vi "RPC Method ThermalChamberController SubscribeChamberStatusUpdated.vi"(8 "error in (no error)":errorcluster, 11 "gRPC service in":refnum<class "ThermalChamberController.lvclass">) -> (0 "error out":errorcluster, 3 "gRPC service out":refnum<class "ThermalChamberController.lvclass">)   [LabVIEW 2020, in "thermal-chamber-controller_server.lvlib" / "ThermalChamberController.lvclass"]
uses:
  ThermalChamberController.lvclass
  support/Stream Data--cluster.ctl
  <vilib>/gRPC/LabVIEW gRPC Library/Shared/grpcId.ctl
  ThermalChamberController.lvclass/ThermalChamberController.ctl
  <vilib>/gRPC/LabVIEW gRPC Library/grpc-lvsupport-release.lvlib
  Program Files (x86)/National Instruments/LabVIEW 2020/examples/DQMH Consortium/DQMH Fundamentals - Thermal Chamber/Libraries/Thermal Chamber Controller_DQMH/Thermal Chamber Controller_DQMH.lvlib
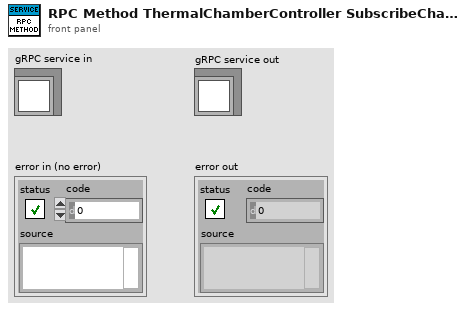
[diagram p1: front panel]
types:
  T1 = typedef "Stream Data--cluster.ctl" = cluster{"gRPCid":T2, "Active":bool, "timeout":i32}
  T2 = typedef "grpc-lvsupport-release.lvlib/grpcId.ctl" = u64
  T3 = typedef "thermal-chamber-controller_server.lvlib/ThermalChamberController.lvclass/Server Internal UEs.ctl" = cluster{"ThermalChamberController StartModule Internal UE":refnum<user-event>, "ThermalChamberController ShowModulePanel Internal UE":refnum<user-event>, "ThermalChamberController HideModulePanel Internal UE":refnum<user-event>, "ThermalChamberController StopModule Internal UE":refnum<user-event>, "ThermalChamberController UpdateSetPoint Internal UE":refnum<user-event>, "ThermalChamberController UpdateRampRate Internal UE":refnum<user-event>, "ThermalChamberController UpdateHeaterState Internal UE":refnum<user-event>, "ThermalChamberController SubscribeChamberStatusUpdated Internal UE":refnum<user-event>, "ThermalChamberController SubscribeSetPointUpdated Internal UE":refnum<user-event>, "ThermalChamberController SubscribeRampRateUpdated Internal UE":refnum<user-event>, "ThermalChamberController SubscribeHeaterStateUpdated Internal UE":refnum<user-event>}
  T4 = typedef "thermal-chamber-controller_server.lvlib/ThermalChamberController.lvclass/Server gRPC UEs.ctl" = cluster{"ThermalChamberController StartModule gRPC UE":refnum<user-event>, "ThermalChamberController ShowModulePanel gRPC UE":refnum<user-event>, "ThermalChamberController HideModulePanel gRPC UE":refnum<user-event>, "ThermalChamberController StopModule gRPC UE":refnum<user-event>, "ThermalChamberController UpdateSetPoint gRPC UE":refnum<user-event>, "ThermalChamberController UpdateRampRate gRPC UE":refnum<user-event>, "ThermalChamberController UpdateHeaterState gRPC UE":refnum<user-event>, "ThermalChamberController SubscribeChamberStatusUpdated gRPC UE":refnum<user-event>, "ThermalChamberController SubscribeSetPointUpdated gRPC UE":refnum<user-event>, "ThermalChamberController SubscribeRampRateUpdated gRPC UE":refnum<user-event>, "ThermalChamberController SubscribeHeaterStateUpdated gRPC UE":refnum<user-event>}
  T5 = typedef "Thermal Chamber Controller_DQMH.lvlib/Broadcast Events--cluster.ctl" = cluster{"Module Did Init":refnum<user-event>, "Status Updated":refnum<user-event>, "Error Reported":refnum<user-event>, "Module Did Stop":refnum<user-event>, "Update Module Execution Status":refnum<user-event>, "Chamber Status Updated":refnum<user-event>, "Set Point Updated":refnum<user-event>, "Ramp Rate Updated":refnum<user-event>, "Heater State Updated":refnum<user-event>}
  T6 = typedef "Thermal Chamber Controller_DQMH.lvlib/Heater State--enum.ctl" = enum16{"Heater Enabled", "Heater Disabled"}
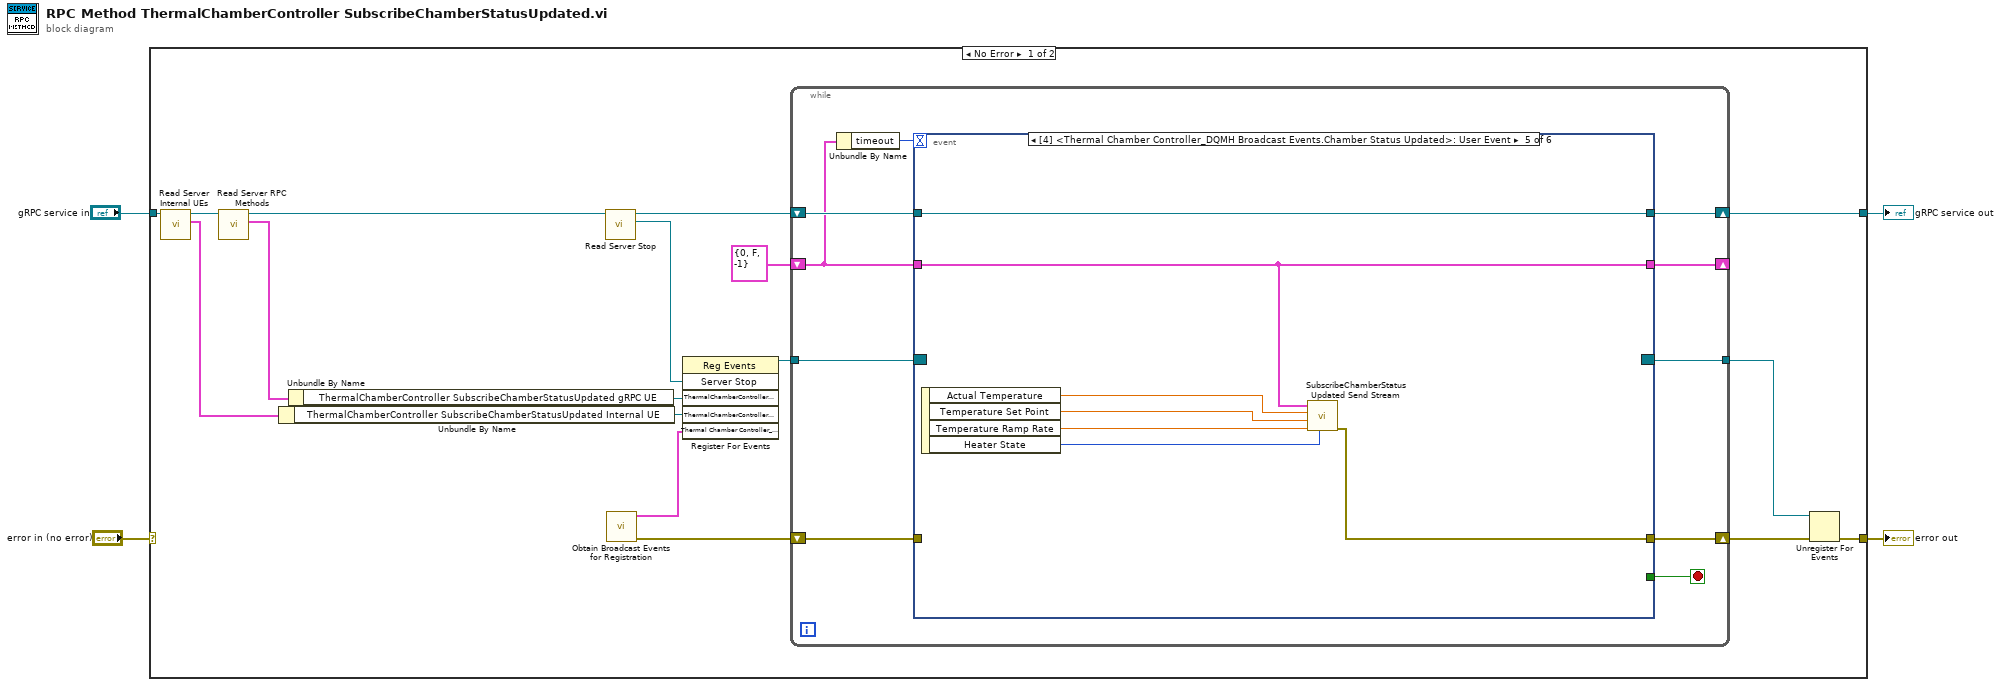
[diagram p0: block diagram]
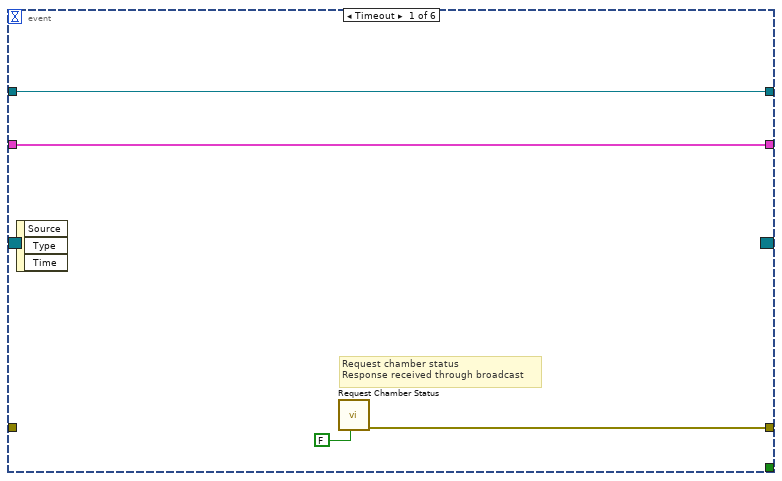
[diagram p2: hidden frame]
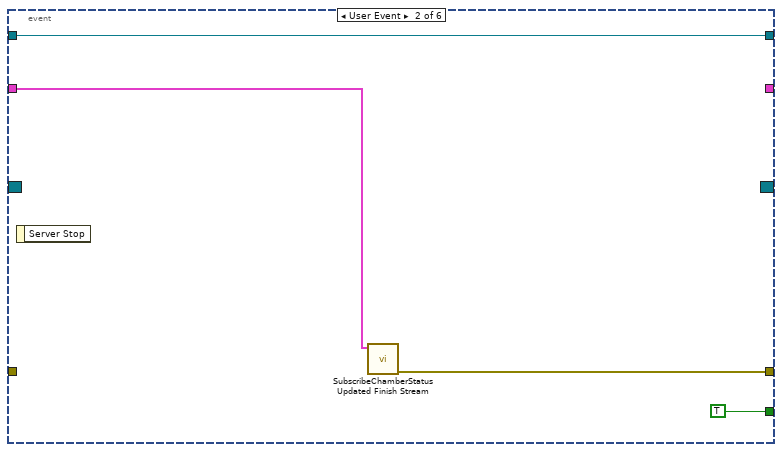
[diagram p3: hidden frame]
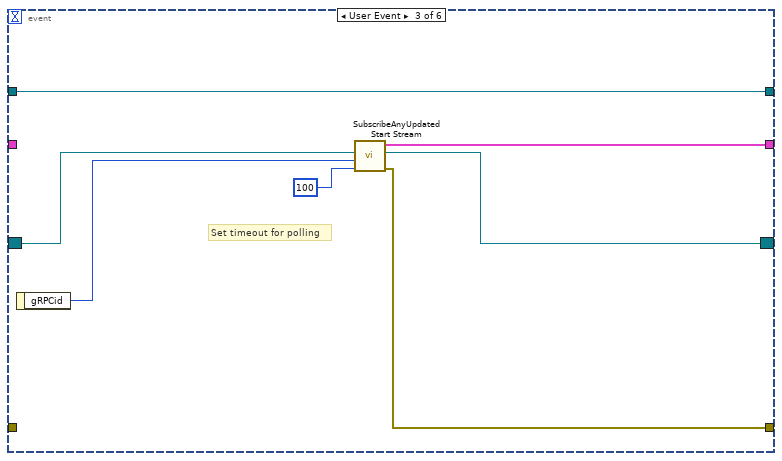
[diagram p4: hidden frame]
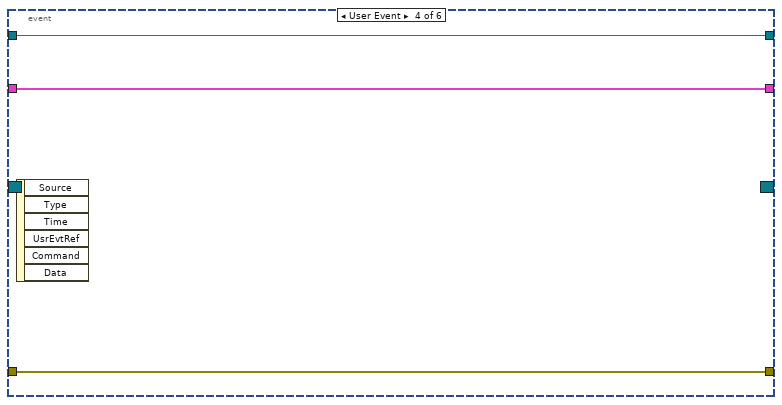
[diagram p5: hidden frame]
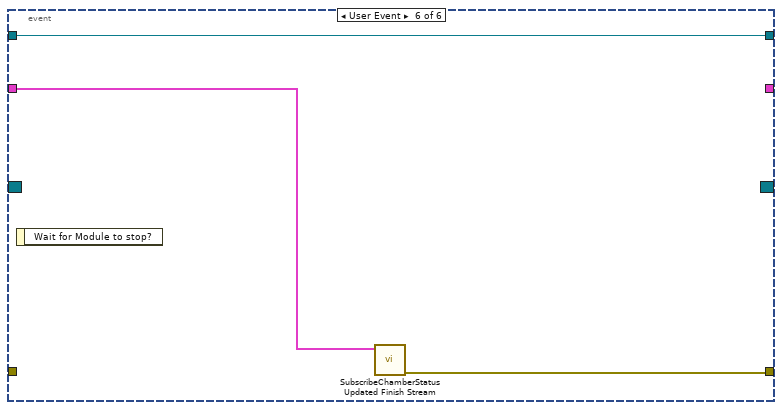
[diagram p6: hidden frame]
diagram:
  n1 = case shown="No Error" "error in (no error)" {
    selector: "error in (no error)" -> [_ w61]
    tunnel: [w16 w61] -> w3
    tunnel: "gRPC service in" -> [w19 w60]
    tunnel: [w8 w60] -> w1
    frame No Error {
      n2 = call "Read Server Internal UEs.vi"("gRPC service in"=w19) -> ("Server Internal UEs"=w12:T3, "gRPC service out"=w18:refnum<class "ThermalChamberController.lvclass">)  [unwired: 8 in, 1 out]
      n3 = call "Read Server RPC Methods.vi"("gRPC service in"=w18) -> ("Server RPC Methods"=w14:T4, "gRPC service out"=w9:refnum<class "ThermalChamberController.lvclass">)  [unwired: 8 in, 1 out]
      n4 = Unbundle By Name ("Unbundle Internal UE")(w12) -> ("ThermalChamberController SubscribeChamberStatusUpdated Internal UE"=w11:refnum<user-event>)
      n5 = Unbundle By Name ("Unbundle gRPC UE")(w14) -> ("ThermalChamberController SubscribeChamberStatusUpdated gRPC UE"=w13:refnum<user-event>)
      n6 = call-dynamic "Read Server Stop.vi"("gRPC service in"=w9) -> ("Server Stop"=w21:refnum<user-event>, "gRPC service out"=w10:refnum<class "ThermalChamberController.lvclass">)  [unwired: 8 in, 1 out]
      n7 = call "Obtain Broadcast Events for Registration.vi"() -> ("error out"=w6:errorcluster, "Thermal Chamber Controller_DQMH Broadcast Events"=w5:T5)  [unwired: 9 in, 1 out]
      n8 = register-events(w21, w13, w11, w5) -> (reference out=w20:refnum<event-registration>)  [unwired: 2 in, 1 out]
      n9 = while {
        tunnel: w20 -> [w31]
        tunnel: [w27] -> w15
        shift-right: [w28] -> w17
        shift-left: w6 -> [w29]
        shift-right: [w25] -> w8
        shift-left: w10 -> [w26]
        shift-right: [w24] -> _
        shift-left: T1 {"gRPCid"=0, "Active"=FALSE, "timeout"=-1} ("Stream Data") -> [w23]
        stop <- w30 stop-if-true
        n10 = Unbundle By Name(w23) -> ("timeout"=w22:i32)
        n11 = event "RPC Method Event Structure" shown="[4] <Thermal Chamber Controller_DQMH Broadcast Events.Chamber Status Updated>: User Event" {
          selector: w31 -> [_ _ w44 _ _ _]
          dyn-events: [_ _ w42 _ _ _] -> w27
          timeout: w22 -> [_ _ _ _ _ _]
          tunnel: [_ TRUE _ _ _ _] -> w30
          tunnel: w29 -> [_ _ _ w49 _ _]
          tunnel: [w32 w37 w41 w49 w50 w57] -> w28
          tunnel: w26 -> [w35 w38 w46 w48 w56 w59]
          tunnel: [w35 w38 w46 w48 w56 w59] -> w25
          tunnel: w23 -> [w34 w36 _ w47 w55 w58]
          tunnel: [w34 _ w45 w47 w55 _] -> w24
          event Timeout {
            # "Request chamber status\nResponse received through broadcast"
            n12 = event-data() -> ()  [unwired: 1 in, 3 out]
            n13 = call "Request Chamber Status.vi"("wait for reply (T)"=FALSE) -> ("error out"=w32:errorcluster)  [unwired: 8 in, 2 out]
          }
          event User Event {
            n14 = event-data() -> ()  [unwired: 1 in, 1 out]
            n15 = call "SubscribeChamberStatusUpdated Finish Stream.vi"("input cluster"=w36) -> ("error out"=w37:errorcluster)  [unwired: 10 in]
          }
          event User Event {
            # "Set timeout for polling"
            n16 = event-data() -> ("gRPCid"=w43:T2)  [unwired: 1 in]
            n17 = call "SubscribeAnyUpdated Start Stream.vi"("timeout"=100, "gRPCid"=w43, "Event Registration Refnum in"=w44) -> ("error out"=w41:errorcluster, "Event Registration Refnum out"=w42:refnum<event-registration>, "Stream Data out"=w45:T1)  [unwired: 6 in]
          }
          event User Event {
            n18 = event-data() -> ()  [unwired: 1 in, 6 out]
          }
          event User Event {
            n19 = event-data() -> ("Actual Temperature"=w54:dbl, "Temperature Set Point"=w53:dbl, "Temperature Ramp Rate"=w52:dbl, "Heater State"=w51:T6)  [unwired: 1 in]
            n20 = call "SubscribeChamberStatusUpdated Send Stream.vi"("Heater State"=w51, "Temperature Ramp Rate"=w52, "Temperature Set Point"=w53, "Actual Temperature"=w54, "input cluster"=w55) -> ("error out"=w50:errorcluster)  [unwired: 6 in]
          }
          event User Event {
            n21 = event-data() -> ()  [unwired: 1 in, 1 out]
            n22 = call "SubscribeChamberStatusUpdated Finish Stream.vi"("input cluster"=w58) -> ("error out"=w57:errorcluster)  [unwired: 10 in]
          }
        }
      }
      n23 = Unregister For Events(event registration refnum=w15, error in=w17) -> (error out=w16:errorcluster)
    }
    frame Error {
    }
  }
  "error out" <- w3
  "gRPC service out" <- w1
